vi "test.recursiveFolderList.vi"() -> ()   [LabVIEW 2017]
panel:
  out "All Files in Dir 2":path[](array[path])
  out "All Files in Dir 2":path[](array[path])
  out "All Files in Dir":path[](array[path])
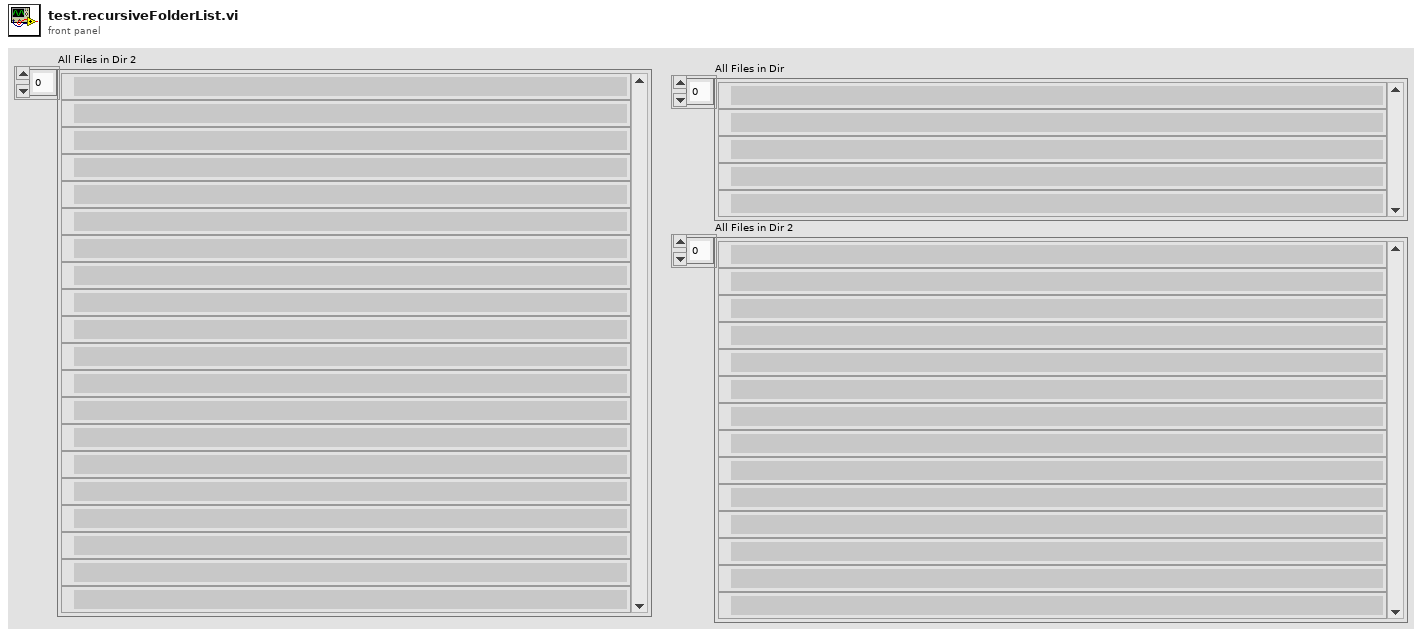
[diagram p1: front panel]
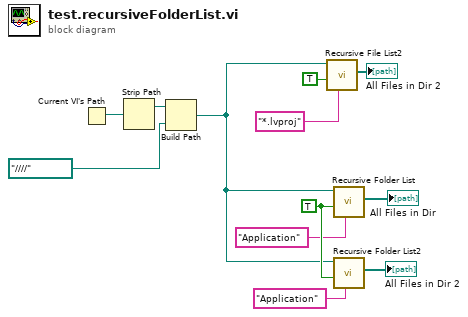
[diagram p0: block diagram]
diagram:
  w8 = TRUE ("Continue Recursing on Error? (F)")
  n1 = Current VI's Path() -> (path=w4:path)
  n2 = Strip Path(path=w4) -> (stripped path=w3:path)  [unwired: 1 out]
  n3 = Build Path(base path=w3, name or relative path=path "../../../../.." ("Folder Path")) -> (appended path=w2:path)
  n4 = call "Recursive File List2.vi"("pattern"="*.lvproj", "Continue Recursing on Error? (F)"=TRUE, "Folder Path"=w2) -> ("All Files in Dir"=→"All Files in Dir 2":path[])  [unwired: 4 in, 4 out]
  n5 = call "Recursive Folder List.vi"("pattern"="Application", "Continue Recursing on Error? (F)"=w8, "Folder Path"=w2) -> ("All Folders"=→"All Files in Dir":path[])  [unwired: 5 in, 3 out]
  n6 = call "Recursive Folder List2.vi"("pattern"="Application", "Continue Recursing on Error? (F)"=w8, "Folder Path"=w2) -> ("All Folders"=→"All Files in Dir 2":path[])  [unwired: 5 in, 3 out]
